vi "GT_Main.vi"() -> ()   [LabVIEW 2018]
doc: "Use this template to build a VI to use as a subVI."
panel:
  out "error out":errorcluster
  out "Alarm History":string[][](array[string])
  out "Manual Allowed":bool
  out "PLC Connected":bool
  out "Alarm Text":string
  out "Home Step Text":string
  out "Left Step Text":string
  out "Right Step Text":string
  out "Cycle Stopping":bool
  out "E-Stop":bool
  out "Alarm":bool
  out "Homed":bool
  out "Manual Mode":bool
  out "Auto Running":bool
  out "Alarm Code":u16
  out "Cycles":u16
  out "Left Count":u16
  out "Right Count":u16
  out "Status":T1
  in  "Exit":bool
  in  "Write":bool
  in  "Target Cycles":u16
  in  "Step Timeout (0.1 s)":u16
  in  "Release Time (0.1 s)":u16
  in  "Vacuum Time (0.1 s)":u16
  out "D107":u16
  in  "Conveyors":bool
  in  "R Vacuum":bool
  in  "R Up":bool
  in  "R Down":bool
  in  "R Rearward":bool
  in  "R Forward":bool
  in  "L Vacuum":bool
  in  "L Up":bool
  in  "L Down":bool
  in  "L Rearward":bool
  in  "L Forward":bool
  in  "Clear Counts":bool
  in  "Reset":bool
  in  "Home":bool
  in  "Stop":bool
  in  "Start":bool
  in  "PLC Port":string
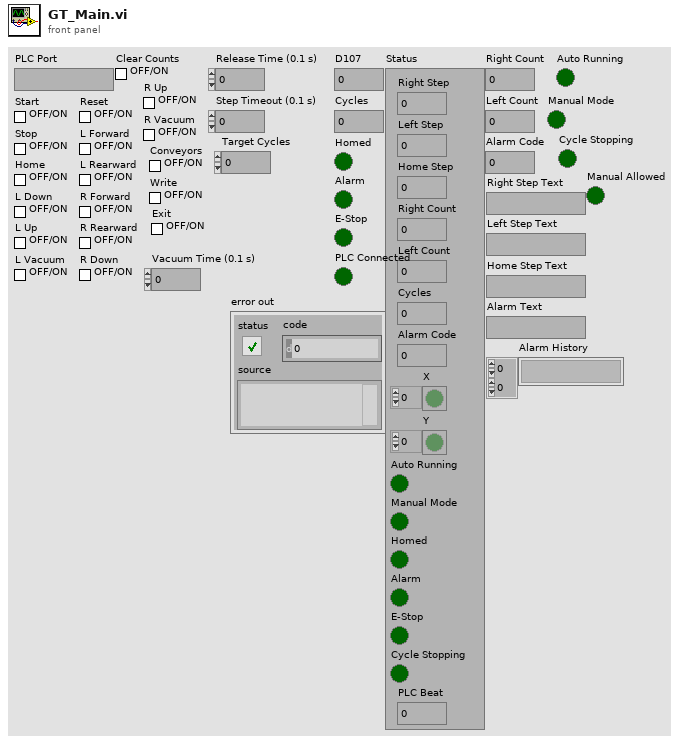
[diagram p1: front panel]
types:
  T1 = cluster{"Right Step":u16, "Left Step":u16, "Home Step":u16, "Right Count":u16, "Left Count":u16, "Cycles":u16, "Alarm Code":u16, "X":bool[], "Y":bool[], "Auto Running":bool, "Manual Mode":bool, "Homed":bool, "Alarm":bool, "E-Stop":bool, "Cycle Stopping":bool, "PLC Beat":u16}
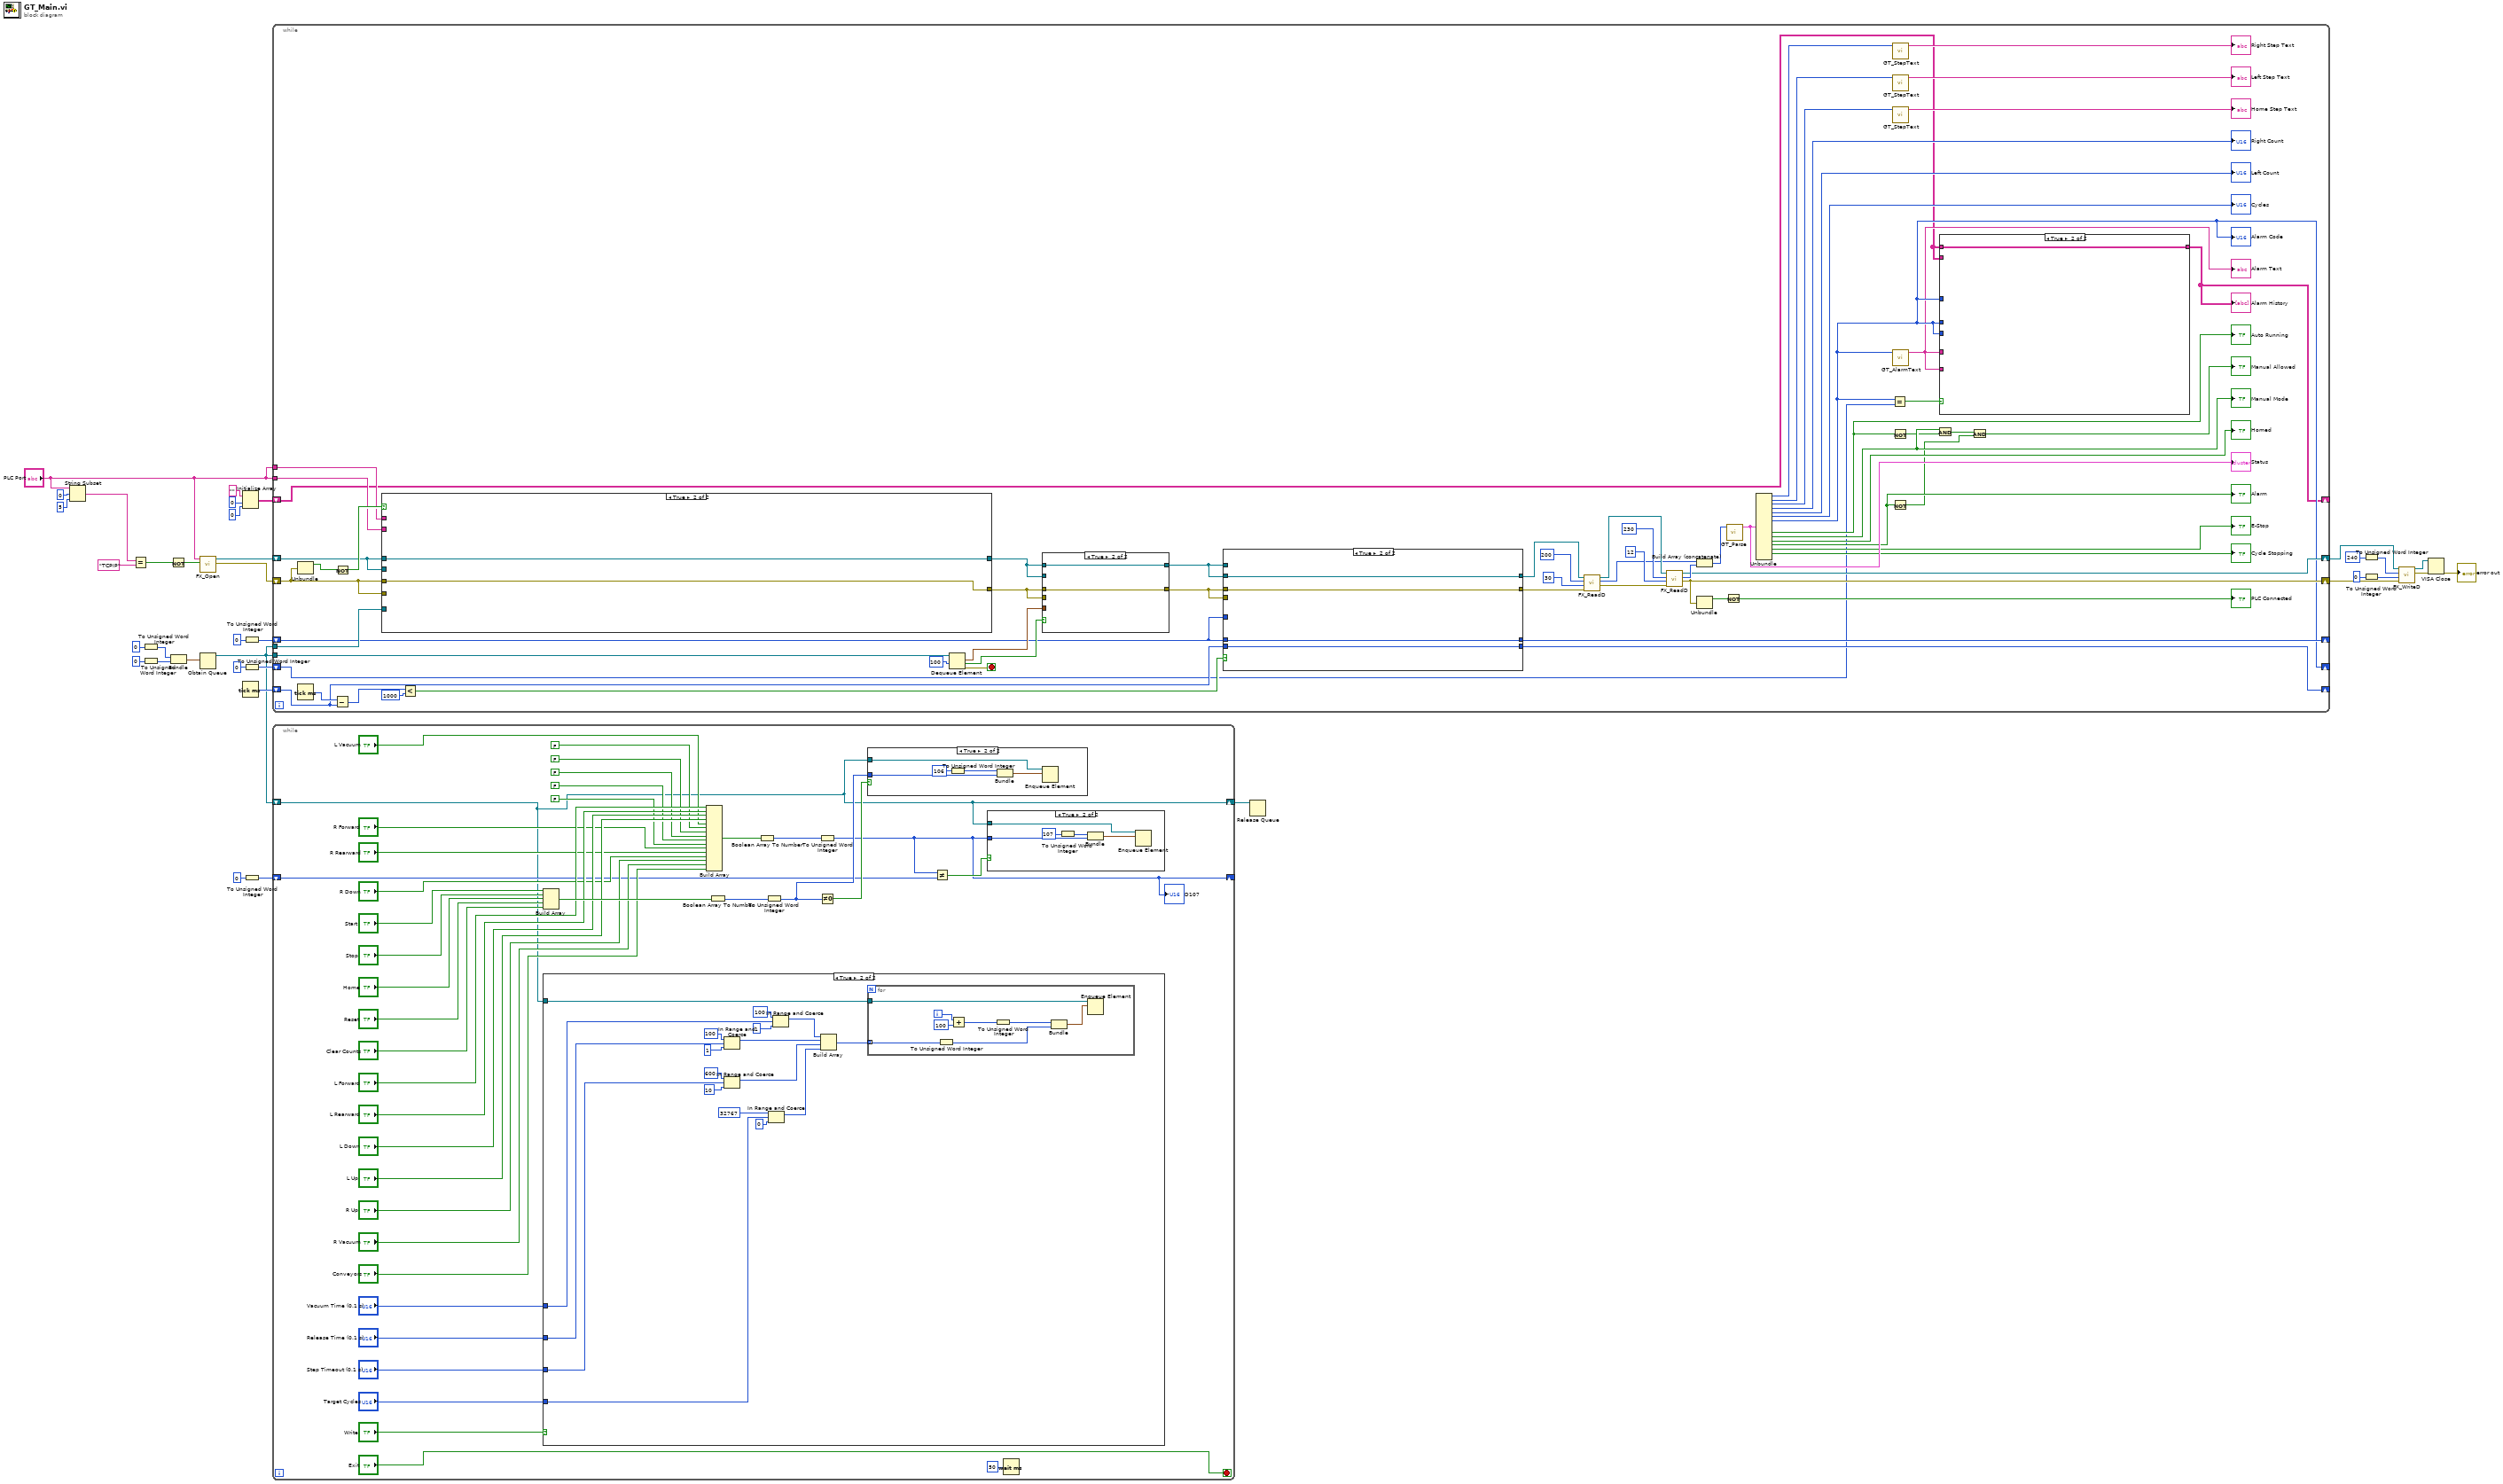
[diagram p0: block diagram]
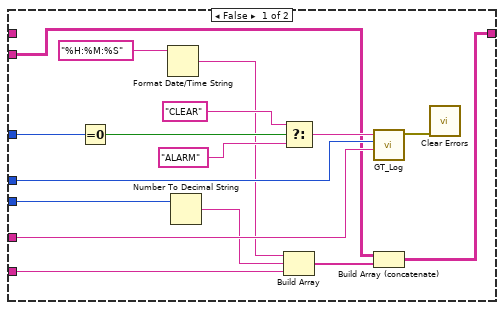
[diagram p2: hidden frame]
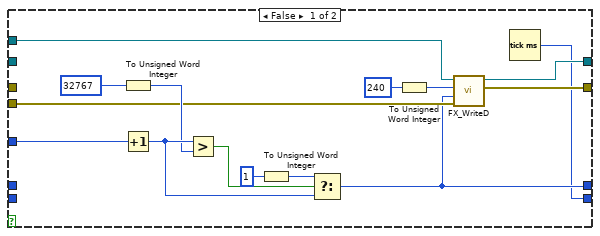
[diagram p3: hidden frame]
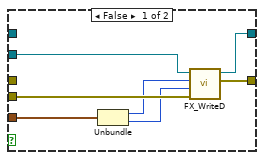
[diagram p4: hidden frame]
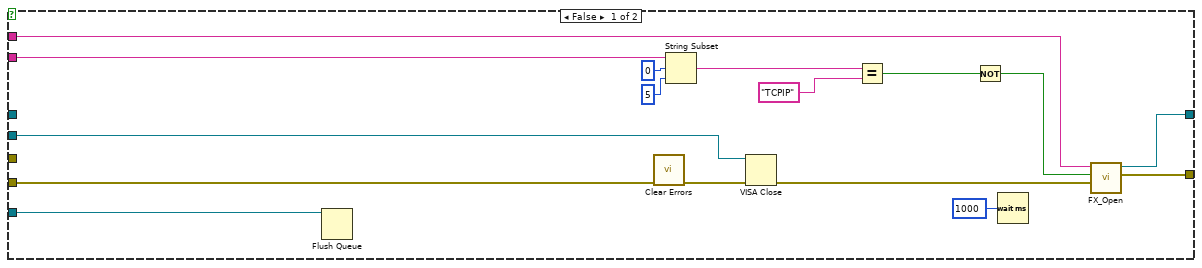
[diagram p5: hidden frame]
diagram:
  n1 = String Subset(string="PLC Port", offset (0)=0, length (rest)=5 ("length (rest)")) -> (substring=w29:string)
  n2 = Equal?(x=w29, y="TCPIP") -> (x = y?=w27:bool)
  n3 = To Unsigned Word Integer(number=0) -> (unsigned 16bit integer=w35:u16)
  n4 = To Unsigned Word Integer(number=0) -> (unsigned 16bit integer=w33:u16)
  n5 = Not(x=w27) -> (.not. x?=w26:bool)
  n6 = Bundle(w35, w33) -> (w32:cluster{u16, u16})  [unwired: 1 in]
  n7 = call "FX_Open.vi"("Serial (COM)?"=w26, "Resource"="PLC Port") -> ("error out"=w21:errorcluster, "VISA out"=w22:refnum<visa-resource-name>)  [unwired: 8 in]
  n8 = Obtain Queue(element data type=w32) -> (queue out=w10:refnum<queue>)  [unwired: 4 in, 2 out]
  n9 = Tick Count (ms)() -> (millisecond timer value=w20:u32)
  n10 = Initialize Array("", 0 ("dimension size"), 0 ("dimension size")) -> (w12:string[][])
  n11 = To Unsigned Word Integer(number=0) -> (unsigned 16bit integer=w18:u16)
  n12 = To Unsigned Word Integer(number=0) -> (unsigned 16bit integer=w16:u16)
  n13 = To Unsigned Word Integer(number=0) -> (unsigned 16bit integer=w24:u16)
  n14 = while {
    shift-right: [w66] -> w7
    shift-left: w22 -> [w96]
    shift-right: [w65] -> w6
    shift-left: w21 -> [w95]
    shift-right: [w78] -> _
    shift-left: w20 -> [w79]
    shift-right: [w80] -> _
    shift-left: w18 -> [w81]
    shift-right: [w40] -> _
    shift-left: w16 -> [w42]
    shift-right: [w37] -> _
    shift-left: w12 -> [w38]
    tunnel: "PLC Port" -> [w99]
    tunnel: "PLC Port" -> [w98]
    tunnel: w10 -> [w97]
    tunnel: w10 -> [w94]
    stop <- w92 stop-if-true
    n15 = Unbundle(w95) -> ("status"=w101:bool)  [unwired: 2 out]
    n16 = Tick Count (ms)() -> (millisecond timer value=w87:u32)
    n17 = Subtract(x=w87, y=w79) -> (x-y=w86:u32)
    n18 = Not(x=w101) -> (.not. x?=w100:bool)
    n19 = case shown="True" w100 {
      tunnel: w95 -> [w162 _]
      tunnel: w96 -> [w161 _]
      tunnel: w99 -> [w158 _]
      tunnel: w98 -> [w157 _]
      tunnel: w97 -> [w149 _]
      tunnel: [w148 w164] -> w89
      tunnel: w96 -> [_ w164]
      tunnel: [w147 w163] -> w88
      tunnel: w95 -> [_ w163]
      frame False {
        n20 = Flush Queue(queue=w149) -> ()  [unwired: 1 in, 3 out]
        n21 = call <vilib>:"Clear Errors.vi"("error in (no error)"=w162) -> ("error out"=w160:errorcluster)  [unwired: 5 in, 1 out]
        n22 = String Subset(string=w157, offset (0)=0, length (rest)=5 ("length (rest)")) -> (substring=w154:string)
        n23 = VISA Close(VISA resource name=w161, error in (no error)=w160) -> (error out=w150:errorcluster)
        n24 = Equal?(x=w154, y="TCPIP") -> (x = y?=w152:bool)
        n25 = Not(x=w152) -> (.not. x?=w151:bool)
        n26 = Wait (ms)(milliseconds to wait=u32 1000) -> ()  [unwired: 1 out]
        n27 = call "FX_Open.vi"("error in (no error)"=w150, "Serial (COM)?"=w151, "Resource"=w158) -> ("error out"=w147:errorcluster, "VISA out"=w148:refnum<visa-resource-name>)  [unwired: 7 in]
      }
      frame True {
      }
    }
    n28 = Less?(x=w86, y=1000) -> (x < y?=w84:bool)
    n29 = Dequeue Element(queue=w94, timeout in ms (-1)=100) -> (element=w90:cluster{u16, u16}, timed out?=w91:bool, error out=w92:errorcluster)  [unwired: 1 in, 1 out]
    n30 = case shown="True" w91 {
      tunnel: w90 -> [w144 _]
      tunnel: w89 -> [w143 _]
      tunnel: w88 -> [w142 _]
      tunnel: [w139 w146] -> w83
      tunnel: w89 -> [_ w146]
      tunnel: [w138 w145] -> w82
      tunnel: w88 -> [_ w145]
      frame False {
        n31 = Unbundle(w144) -> (w141:u16, w140:u16)
        n32 = call "FX_WriteD.vi"("error in (no error)"=w142, "Value"=w140, "D"=w141, "VISA in"=w143) -> ("error out"=w138:errorcluster, "VISA out"=w139:refnum<visa-resource-name>)  [unwired: 6 in]
      }
      frame True {
      }
    }
    n33 = case shown="True" w84 {
      tunnel: w81 -> [w133 _]
      tunnel: w83 -> [w125 _]
      tunnel: w82 -> [w124 _]
      tunnel: [w122 w137] -> w77
      tunnel: w83 -> [_ w137]
      tunnel: [w121 w136] -> w76
      tunnel: w82 -> [_ w136]
      tunnel: [w120 w135] -> w80
      tunnel: w81 -> [_ w135]
      tunnel: [w119 w134] -> w78
      tunnel: w79 -> [_ w134]
      frame False {
        n34 = To Unsigned Word Integer(number=32767) -> (unsigned 16bit integer=w130:u16)
        n35 = Increment(x=w133) -> (x+1=w131:u16)
        n36 = Greater?(x=w131, y=w130) -> (0:w129:bool)
        n37 = To Unsigned Word Integer(number=1) -> (unsigned 16bit integer=w127:u16)
        n38 = Select(t=w127, s=w129, f=w131) -> (s? t:f=w120:u16)
        n39 = To Unsigned Word Integer(number=240) -> (unsigned 16bit integer=w123:u16)
        n40 = call "FX_WriteD.vi"("error in (no error)"=w124, "Value"=w120, "D"=w123, "VISA in"=w125) -> ("error out"=w121:errorcluster, "VISA out"=w122:refnum<visa-resource-name>)  [unwired: 6 in]
        n41 = Tick Count (ms)() -> (millisecond timer value=w119:u32)
      }
      frame True {
      }
    }
    n42 = call "FX_ReadD.vi"("error in (no error)"=w76, "Count"=u16 30, "D"=u16 200, "VISA in"=w77) -> ("error out"=w72:errorcluster, "Words"=w69:u16[], "VISA out"=w73:refnum<visa-resource-name>)  [unwired: 5 in]
    n43 = call "FX_ReadD.vi"("error in (no error)"=w72, "Count"=u16 12, "D"=u16 230, "VISA in"=w73) -> ("error out"=w65:errorcluster, "Words"=w68:u16[], "VISA out"=w66:refnum<visa-resource-name>)  [unwired: 5 in]
    n44 = Build Array (concatenate)(w69, w68) -> (w67:u16[])
    n45 = Unbundle(w65) -> ("status"=w48:bool)  [unwired: 2 out]
    n46 = Not(x=w48) -> (.not. x?=→"PLC Connected":bool)
    n47 = call "GT_Parse.vi"("Words"=w67) -> ("Status"=w64:T1)  [unwired: 10 in]
    "Status" <- w64
    n48 = Unbundle(w64) -> ("Right Step"=w54:u16, "Left Step"=w52:u16, "Home Step"=w50:u16, "Right Count"=→"Right Count":u16, "Left Count"=→"Left Count":u16, "Cycles"=→"Cycles":u16, "Alarm Code"=w40:u16, "Auto Running"=w60:bool, "Manual Mode"=w59:bool, "Homed"=→"Homed":bool, "Alarm"=w57:bool, "E-Stop"=→"E-Stop":bool, "Cycle Stopping"=→"Cycle Stopping":bool)  [unwired: 3 out]
    "Alarm Code" <- w40
    "Auto Running" <- w60
    "Manual Mode" <- w59
    "Alarm" <- w57
    n49 = Equal?(x=w40, y=w42) -> (x = y?=w41:bool)
    n50 = Not(x=w60) -> (.not. x?=w46:bool)
    n51 = Not(x=w57) -> (.not. x?=w44:bool)
    n52 = call "GT_StepText.vi"("Step"=w54) -> ("Step Text"=→"Right Step Text":string)  [unwired: 10 in]
    n53 = call "GT_StepText.vi"("Step"=w52) -> ("Step Text"=→"Left Step Text":string)  [unwired: 10 in]
    n54 = call "GT_StepText.vi"("Step"=w50) -> ("Step Text"=→"Home Step Text":string)  [unwired: 10 in]
    n55 = call "GT_AlarmText.vi"("Alarm Code"=w40) -> ("Alarm Text"=w39:string)  [unwired: 10 in]
    "Alarm Text" <- w39
    n56 = And(x=w59, y=w46) -> (x .and. y?=w45:bool)
    n57 = case shown="True" w41 {
      tunnel: w40 -> [w117 _]
      tunnel: w40 -> [w112 _]
      tunnel: w39 -> [w111 _]
      tunnel: w40 -> [w108 _]
      tunnel: w39 -> [w105 _]
      tunnel: w38 -> [w104 _]
      tunnel: [w102 w118] -> w37
      tunnel: w38 -> [_ w118]
      frame False {
        n58 = Equal To 0?(x=w117) -> (x = 0?=w116:bool)
        n59 = Format Date/Time String(time format string (%c)="%H:%M:%S") -> (date/time string=w107:string)  [unwired: 2 in]
        n60 = Number To Decimal String(number=w108) -> (decimal integer string=w106:string)  [unwired: 1 in]
        n61 = Select(t="CLEAR", s=w116, f="ALARM") -> (s? t:f=w113:string)
        n62 = Build Array(w107, w106, w105) -> (w103:string[])
        n63 = call "GT_Log.vi"("Text"=w111, "Code"=w112, "Event"=w113) -> ("error out"=w110:errorcluster)  [unwired: 8 in]
        n64 = Build Array (concatenate)(w104, w103) -> (w102:string[][])
        n65 = call <vilib>:"Clear Errors.vi"("error in (no error)"=w110) -> ()  [unwired: 5 in, 2 out]
      }
      frame True {
      }
    }
    "Alarm History" <- w37
    n66 = And(x=w45, y=w44) -> (x .and. y?=→"Manual Allowed":bool)
  }
  n67 = while {
    shift-right: [w167] -> w23
    shift-left: w10 -> [w167]
    shift-right: [w173] -> _
    shift-left: w24 -> [w175]
    stop <- "Exit" stop-if-true
    n68 = Build Array("Start", "Stop", "Home", "Reset", "Clear Counts") -> (w197:bool[])
    n69 = case shown="True" "Write" {
      tunnel: "Vacuum Time (0.1 s)" -> [_ w220]
      tunnel: "Release Time (0.1 s)" -> [_ w217]
      tunnel: "Step Timeout (0.1 s)" -> [_ w214]
      tunnel: "Target Cycles" -> [_ w211]
      tunnel: w167 -> [_ w203]
      frame False {
      }
      frame True {
        n70 = In Range and Coerce(upper limit=u16 100, x=w217, lower limit=u16 1) -> (coerced(x)=w207:u16)  [unwired: 1 out]
        n71 = In Range and Coerce(upper limit=u16 600, x=w214, lower limit=u16 10) -> (coerced(x)=w206:u16)  [unwired: 1 out]
        n72 = In Range and Coerce(upper limit=u16 32767, x=w211, lower limit=u16 0) -> (coerced(x)=w205:u16)  [unwired: 1 out]
        n73 = In Range and Coerce(upper limit=u16 100, x=w220, lower limit=u16 1) -> (coerced(x)=w208:u16)  [unwired: 1 out]
        n74 = Build Array(w208, w207, w206, w205) -> (w204:u16[])
        n75 = for {
          tunnel: w204 -> [w228] mode=indexing
          tunnel: w203 -> [w222]
          i -> [w227]
          n76 = To Unsigned Word Integer(number=w228) -> (unsigned 16bit integer=w223:u16)
          n77 = Add(x=w227, y=100) -> (x+y=w225:i32)
          n78 = To Unsigned Word Integer(number=w225) -> (unsigned 16bit integer=w224:u16)
          n79 = Bundle(w224, w223) -> (w221:cluster{u16, u16})  [unwired: 1 in]
          n80 = Enqueue Element(queue=w222, element=w221) -> ()  [unwired: 2 in, 3 out]
        }
      }
    }
    n81 = Build Array("L Forward", "L Rearward", "L Down", "L Up", "L Vacuum", FALSE, FALSE, FALSE, FALSE, FALSE, "R Forward", "R Rearward", "R Down", "R Up", "R Vacuum", "Conveyors") -> (w177:bool[])
    n82 = Boolean Array To Number(Boolean array=w197) -> (number=w196:u32)
    n83 = Boolean Array To Number(Boolean array=w177) -> (number=w176:u32)
    n84 = To Unsigned Word Integer(number=w196) -> (unsigned 16bit integer=w194:u16)
    n85 = To Unsigned Word Integer(number=w176) -> (unsigned 16bit integer=w173:u16)
    "D107" <- w173
    n86 = Not Equal To 0?(x=w194) -> (x != 0?=w195:bool)
    n87 = case shown="True" w195 {
      tunnel: w194 -> [_ w236]
      tunnel: w167 -> [_ w235]
      frame False {
      }
      frame True {
        n88 = To Unsigned Word Integer(number=106) -> (unsigned 16bit integer=w237:u16)
        n89 = Bundle(w237, w236) -> (w234:cluster{u16, u16})  [unwired: 1 in]
        n90 = Enqueue Element(queue=w235, element=w234) -> ()  [unwired: 2 in, 3 out]
      }
    }
    n91 = Not Equal?(x=w173, y=w175) -> (x != y?=w174:bool)
    n92 = case shown="True" w174 {
      tunnel: w173 -> [_ w231]
      tunnel: w167 -> [_ w230]
      frame False {
      }
      frame True {
        n93 = To Unsigned Word Integer(number=107) -> (unsigned 16bit integer=w232:u16)
        n94 = Bundle(w232, w231) -> (w229:cluster{u16, u16})  [unwired: 1 in]
        n95 = Enqueue Element(queue=w230, element=w229) -> ()  [unwired: 2 in, 3 out]
      }
    }
    n96 = Wait (ms)(milliseconds to wait=u32 50) -> ()  [unwired: 1 out]
  }
  n97 = Release Queue(queue=w23) -> ()  [unwired: 2 in, 3 out]
  n98 = To Unsigned Word Integer(number=240) -> (unsigned 16bit integer=w5:u16)
  n99 = To Unsigned Word Integer(number=0) -> (unsigned 16bit integer=w4:u16)
  n100 = call "FX_WriteD.vi"("error in (no error)"=w6, "Value"=w4, "D"=w5, "VISA in"=w7) -> ("error out"=w2:errorcluster, "VISA out"=w3:refnum<visa-resource-name>)  [unwired: 6 in]
  n101 = VISA Close(VISA resource name=w3, error in (no error)=w2) -> (error out=→"error out":errorcluster)
